vi "set Trace Mode.vi"(8 "error in (no error)":errorcluster, 9 "Trace Index":u32=1 min=1, 10 "Trace Mode":T1, 11 "FSV-40N in":refnum<class "FSV-40N.lvclass">) -> (0 "error out":errorcluster, 3 "FSV-40N out":refnum<class "FSV-40N.lvclass">)   [LabVIEW 2023, in "Spectrum Analyzer.lvlib" / "FSV-40N.lvclass"]
uses:
  FSV-40N.lvclass
  FSV-40N.lvclass/FSV-40N.ctl
  TYPE DEFINITION/TYPE Display Trace Mode Select.ctl
  Spectrum Analyzer.lvlib
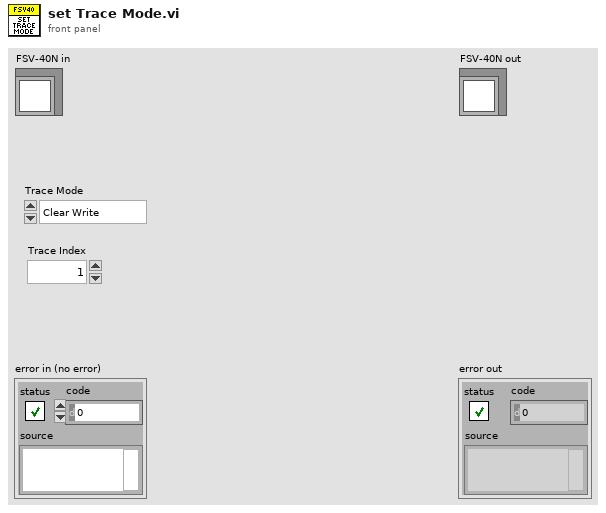
[diagram p1: front panel]
types:
  T1 = typedef "Spectrum Analyzer.lvlib/TYPE Display Trace Mode Select.ctl" = enum16{"Clear Write", "Max Hold", "Min Hold", "Average", "View"}
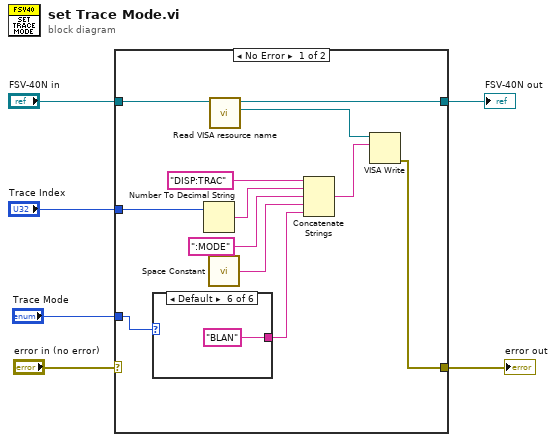
[diagram p0: block diagram]
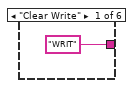
[diagram p2: hidden frame]
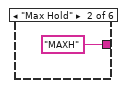
[diagram p3: hidden frame]
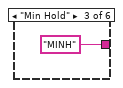
[diagram p4: hidden frame]
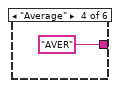
[diagram p5: hidden frame]
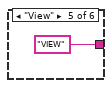
[diagram p6: hidden frame]
diagram:
  n1 = case shown="No Error" "error in (no error)" {
    selector: "error in (no error)" -> [_ w26]
    tunnel: "FSV-40N in" -> [w18 w25]
    tunnel: "Trace Index" -> [w17 _]
    tunnel: "Trace Mode" -> [w12 _]
    tunnel: [w8 w25] -> w2
    tunnel: [w7 w26] -> w1
    frame No Error {
      n2 = case shown="Default" w12 {
        tunnel: ["WRIT" "MAXH" "MINH" "AVER" "VIEW" "BLAN"] -> w11
        frame "Clear Write" {
        }
        frame "Max Hold" {
        }
        frame "Min Hold" {
        }
        frame "Average" {
        }
        frame "View" {
        }
        frame Default {
        }
      }
      n3 = Number To Decimal String(number=w17) -> (decimal integer string=w15:string)  [unwired: 1 in]
      n4 = call <vilib>:"Space Constant.vi"() -> ("String"=w13:string)
      n5 = call "Read VISA resource name.vi"("FSV-40N in"=w18) -> ("VISA resource name"=w9:refnum<visa-resource-name>, "FSV-40N out"=w8:refnum<class "FSV-40N.lvclass">)  [unwired: 8 in, 1 out]
      n6 = Concatenate Strings("DISP:TRAC" ("write buffer"), w15, ":MODE" ("string"), w13, w11) -> (w10:string)
      n7 = VISA Write(VISA resource name=w9, write buffer=w10) -> (error out=w7:errorcluster)  [unwired: 1 in, 2 out]
    }
    frame Error {
    }
  }
  "error out" <- w1
  "FSV-40N out" <- w2
